vi "_Engine Core.vi"(11 "Cluster":T3) -> ()   [LabVIEW 2012]
uses:
  <vilib>/Utility/miscctls.llb/LVPositionTypeDef.ctl
  Move Speed.ctl
panel:
  out "Numeric":i32
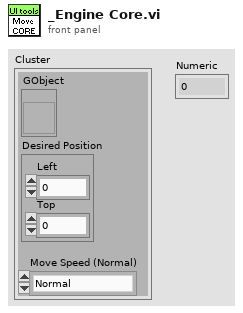
[diagram p1: front panel]
types:
  T1 = typedef "LVPositionTypeDef.ctl" = cluster{"Left":i32, "Top":i32}
  T2 = typedef "Move Speed.ctl" = enum16{"Normal", "Fast", "Slow", "Instantaneous"}
  T3 = cluster{"GObject":refnum<vi>, "Desired Position":T1, "Move Speed (Normal)":T2}
  T4 = typedef "LVBoundsTypeDef.ctl" = cluster{"Width":u32, "Height":u32}
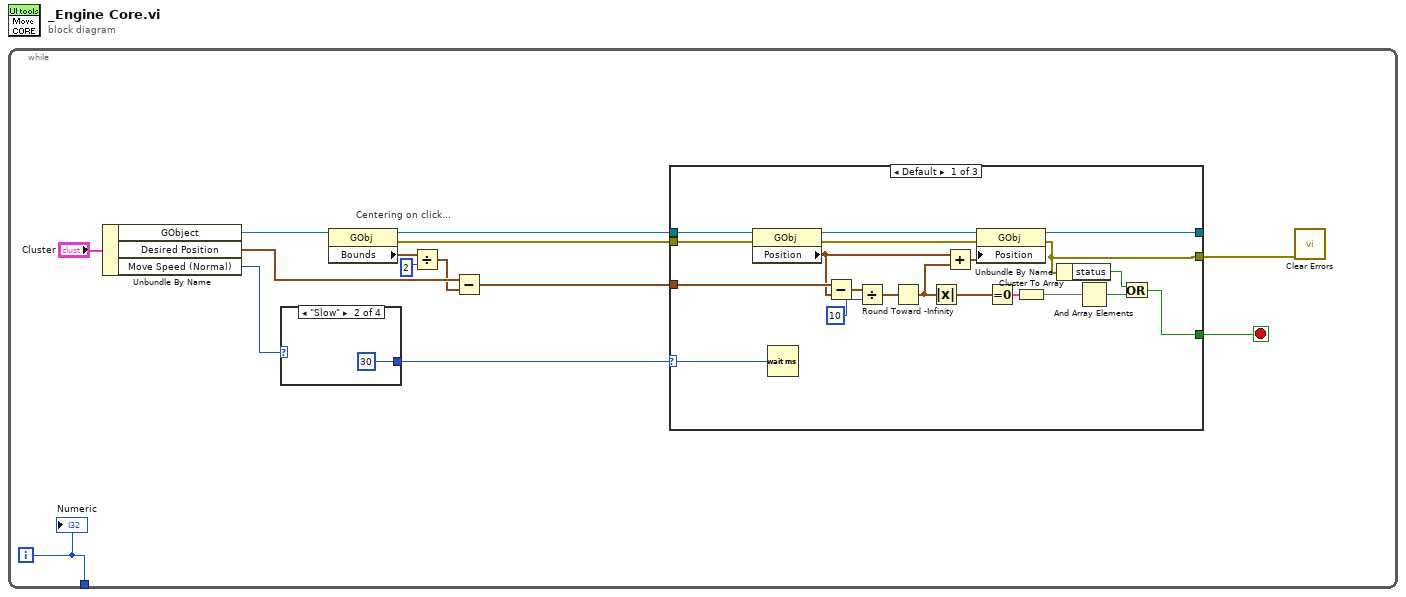
[diagram p0: block diagram]
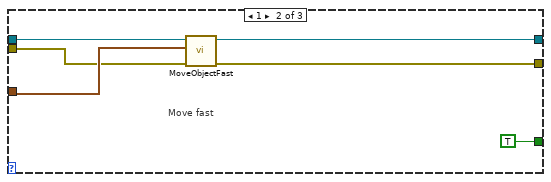
[diagram p2: hidden frame]
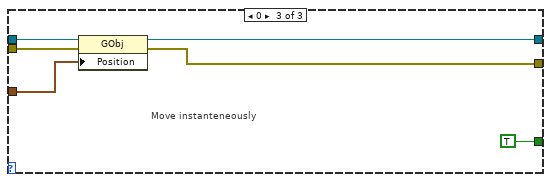
[diagram p3: hidden frame]
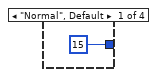
[diagram p4: hidden frame]
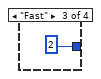
[diagram p5: hidden frame]
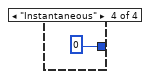
[diagram p6: hidden frame]
diagram:
  n1 = while {
    tunnel: [w1] -> _
    i -> [w1]
    stop <- w2 stop-if-true
    # "Centering on click..."
    n2 = Unbundle By Name("Cluster") -> ("GObject"=w13:refnum<vi>, "Desired Position"=w12:T1, "Move Speed (Normal)"=w11:T2)
    n3 = case shown="\"Slow\"" w11 {
      tunnel: [u32 15 ("Sliding Speed (40)") u32 30 ("Sliding Speed (40)") u32 2 ("Sliding Speed (40)") u32 0 ("Sliding Speed (40)")] -> w5
      frame "Normal", Default {
      }
      frame "Slow" {
      }
      frame "Fast" {
      }
      frame "Instantaneous" {
      }
    }
    n4 = property class="GObj"(reference=w13) -> (reference out=w10:refnum<vi>, error out=w9:errorcluster, "Bounds"=w8:T4)  [unwired: 1 in]
    n5 = Divide(x=w8, y=2) -> (x/y=w6:cluster{"Width":dbl, "Height":dbl})
    n6 = Subtract(x=w12, y=w6) -> (x-y=w3:cluster{dbl, dbl})
    n7 = case shown="Default" w5 {
      selector: w5 -> [w30 _ _]
      tunnel: w10 -> [w34 w40 w44]
      tunnel: w9 -> [w33 w38 w45]
      tunnel: w3 -> [w32 w39 w43]
      tunnel: [w31 w37 w46] -> _
      tunnel: [w29 w36 w42] -> w4
      tunnel: [w28 TRUE TRUE] -> w2
      frame Default {
        n8 = property class="GObj"(reference=w34, error in=w33) -> (reference out=w27:refnum<vi>, error out=w21:errorcluster, "Position"=w24:T1)
        n9 = Wait (ms)(milliseconds to wait=w30) -> ()  [unwired: 1 out]
        n10 = Subtract(x=w32, y=w24) -> (x-y=w23:cluster{dbl, dbl})
        n11 = Divide(x=w23, y=10) -> (x/y=w17:cluster{dbl, dbl})
        n12 = Round Toward -Infinity(1:w17) -> (0:w16:cluster{dbl, dbl})
        n13 = Absolute Value(x=w16) -> (abs(x)=w15:cluster{dbl, dbl})
        n14 = Add(x=w24, y=w16) -> (x+y=w18:cluster{dbl, dbl})
        n15 = property class="GObj"(reference=w27, error in=w21, "Position"=w18) -> (reference out=w31:refnum<vi>, error out=w29:errorcluster)
        n16 = Equal To 0?(x=w15) -> (x = 0?=w25:cluster{bool, bool})
        n17 = Cluster To Array(cluster=w25) -> (array=w26:bool[])
        n18 = Unbundle By Name(w29) -> ("status"=w19:bool)
        n19 = And Array Elements(Boolean array=w26) -> (logical AND=w20:bool)
        n20 = Or(x=w19, y=w20) -> (x .or. y?=w28:bool)
      }
      frame 1 {
        # "Move fast"
        n21 = call "MoveObjectFast.vi"("error in"=w38, "Position"=w39, "GObj Refnum"=w40) -> ("error out"=w36:errorcluster, "GObj Refnum dup"=w37:refnum<vi>)  [unwired: 7 out]
      }
      frame 0 {
        # "Move instanteneously"
        n22 = property class="GObj"(reference=w44, error in=w45, "Position"=w43) -> (reference out=w46:refnum<vi>, error out=w42:errorcluster)
      }
    }
    n23 = call <vilib>:"Clear Errors.vi"("error in (no error)"=w4) -> ()  [unwired: 7 out]
    "Numeric" <- w1
  }
